vi "Read Queue Items.vi"(11 "Protected Actor Handle in":refnum<class "Protected Actor Handle.lvclass">) -> (1 "Message Names":string[](array[string]), 2 "# Messages in queue":i32)   [LabVIEW 2020, in "Actor Framework.lvlib" / "Protected Actor Handle.lvclass"]
doc: "Reads queue information from the actor message queues, useful for display in a debugger.\n\nReturns Count and Message class IDs."
uses:
  Protected Actor Handle.lvclass
  Protected Actor Handle.lvclass/Protected Actor Handle.ctl
  Message Enqueuer/Message Enqueuer.lvclass
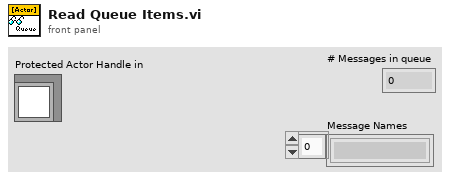
[diagram p1: front panel]
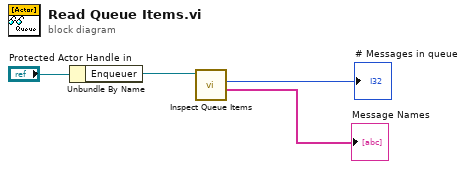
[diagram p0: block diagram]
diagram:
  n1 = Unbundle By Name("Protected Actor Handle in") -> ("Enqueuer"=w3:refnum<class "Message Enqueuer.lvclass">)
  n2 = call "Inspect Queue Items.vi"("Message Enqueuer in"=w3) -> ("Message Names"=→"Message Names":string[], "# Messages in queue"=→"# Messages in queue":i32)  [unwired: 7 in, 2 out]
